vi "Scroll-Hmove.vi"(8 "error in (no error)":errorcluster, 9 "New coordinate":T1, 11 "Gviewer in":refnum<class "Gviewer.lvclass">) -> (0 "error out":errorcluster, 3 "Gviewer out":refnum<class "Gviewer.lvclass">)   [LabVIEW 2020, in "Sgraph_lib_V1.lvlib" / "Gviewer.lvclass"]
doc: "Andre Koelewijn, 14 feb 2021\n\nThis VI perform the actual horizontal move in respect to the position where the mouse was clicked."
uses:
  Gviewer.lvclass
  <vilib>/Utility/miscctls.llb/LVPoint32TypeDef.ctl
  Gviewer.lvclass/Gviewer.ctl
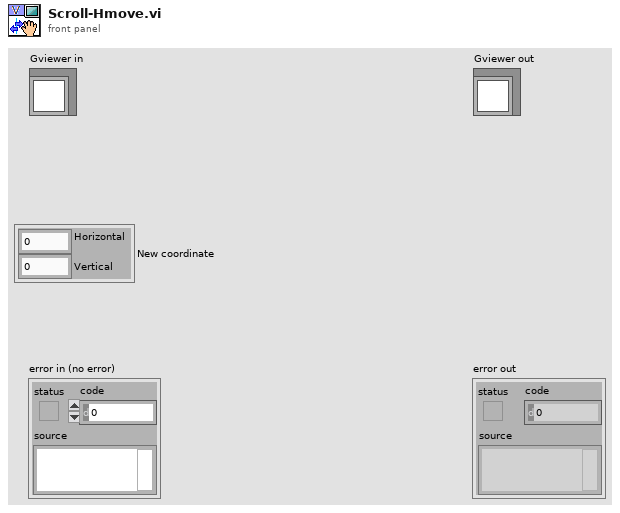
[diagram p1: front panel]
types:
  T1 = typedef "LVPoint32TypeDef.ctl" = cluster{"Horizontal":i32, "Vertical":i32}
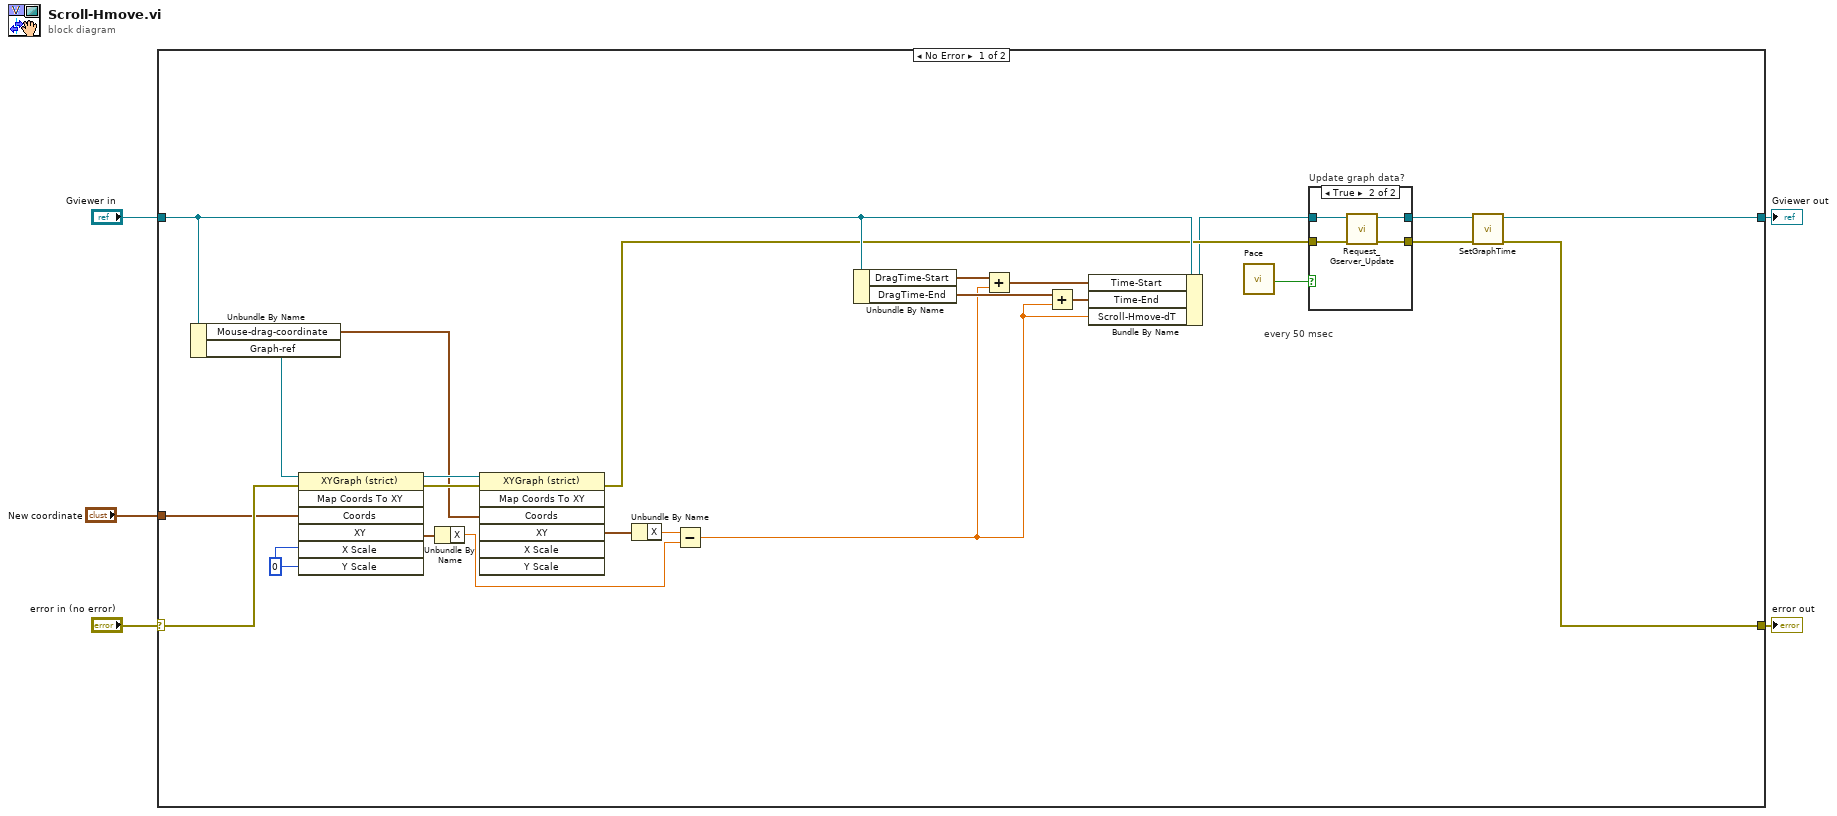
[diagram p0: block diagram]
diagram:
  n1 = case shown="No Error" "error in (no error)" {
    selector: "error in (no error)" -> [w27 w37]
    tunnel: [w8 w37] -> w4
    tunnel: [w6 w36] -> w2
    tunnel: "Gviewer in" -> [w18 w36]
    tunnel: "New coordinate" -> [w26 _]
    frame No Error {
      w29 = 0 ("Y Scale")
      # "every 50 msec"
      n2 = Unbundle By Name(w18) -> ("Mouse-drag-coordinate"=w22:T1, "Graph-ref"=w21:refnum<vi>)
      n3 = invoke class="XYGraph (strict)" method="Map Coords To XY"(reference=w21, error in=w27, "Coords"=w26, "X Scale"=w29, "Y Scale"=w29) -> (reference out=w23:refnum<vi>, error out=w24:errorcluster, "XY"=w28:cluster{"X":dbl, "Y":dbl})  [unwired: 2 in, 4 out]
      n4 = Unbundle By Name(w28) -> ("X"=w19:dbl)
      n5 = invoke class="XYGraph (strict)" method="Map Coords To XY"(reference=w23, error in=w24, "Coords"=w22) -> (error out=w17:errorcluster, "XY"=w25:cluster{"X":dbl, "Y":dbl})  [unwired: 4 in, 5 out]
      n6 = Unbundle By Name(w25) -> ("X"=w20:dbl)
      n7 = Subtract(x=w20, y=w19) -> (x-y=w11:dbl)
      n8 = Unbundle By Name(w18) -> ("DragTime-Start"=w16:timestamp, "DragTime-End"=w15:timestamp)
      n9 = Add(x=w16, y=w11) -> (x+y=w14:timestamp)
      n10 = Add(x=w15, y=w11) -> (x+y=w13:timestamp)
      n11 = Bundle By Name(cluster=w18, "Time-Start"=w14, "Time-End"=w13, "Scroll-Hmove-dT"=w11) -> (w7:refnum<class "Gviewer.lvclass">)
      n12 = call "Pace"() -> ("Time has Elapsed"=w12:bool)  [unwired: 12 in, 7 out]
      n13 = case "Update graph data?" shown="True" w12 {
        tunnel: w17 -> [w31 w35]
        tunnel: [w31 w34] -> w10
        tunnel: w7 -> [w30 w33]
        tunnel: [w30 w32] -> w9
        frame False {
        }
        frame True {
          n14 = call "Request_Gserver_Update.vi"("error in (no error)"=w35, "Gviewer in"=w33) -> ("error out"=w34:errorcluster, "Gviewer out"=w32:refnum<class "Gviewer.lvclass">)  [unwired: 8 in]
        }
      }
      n15 = call "SetGraphTime.vi"("error in (no error)"=w10, "Gviewer in"=w9) -> ("error out"=w8:errorcluster, "Gviewer out"=w6:refnum<class "Gviewer.lvclass">)  [unwired: 8 in]
    }
    frame Error {
    }
  }
  "error out" <- w4
  "Gviewer out" <- w2
